vi "VHistFile - Open or Create File.vi"(6 "create if doesn't exist (F)":bool, 8 "error in":errorcluster, 9 "deny mode (2)":T1(ring)=enum."deny none", 10 "open mode (0)":T2(ring), 11 "file path":path) -> (0 "error out":errorcluster, 3 "file refnum":refnum<file>)   [LabVIEW 2021]
doc: "::: CalcExpress Toolkit :::\nCopyright (c) 2000-2026 Konstantin Shifershteyn. All rights reserved."
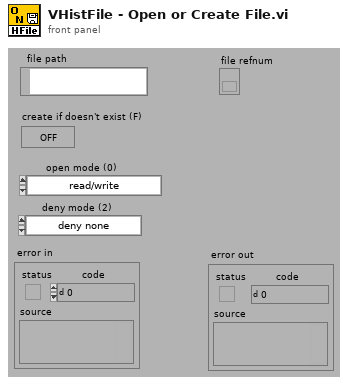
[diagram p1: front panel]
types:
  T1 = enum16{"deny read/write", "deny write-only", "deny none"}
  T2 = enum16{"read/write", "read-only", "write-only", "write-only (truncate)"}
  T3 = enum16{"open", "replace", "create", "open or create", "replace or create", "replace or create with confirmation"}
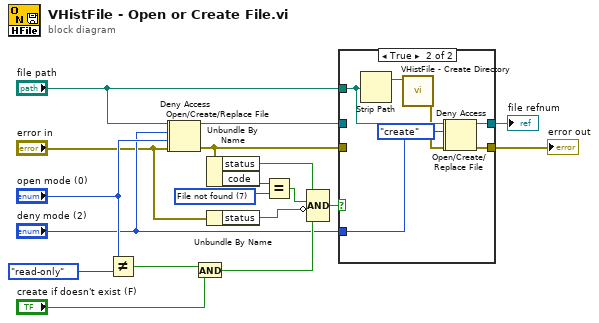
[diagram p0: block diagram]
diagram:
  w15 = u16 7 items=["No error", "Argument error", "Memory is full", "Out of zone", "End of file", "File already open", "Generic file I/O error", "File not found", "File permission error", "Disk is full", "Duplicate path", "Too many files open", "System feature not enabled", "Resource file not found", "Cannot add resource", "Resource not found", "Image not found", "Image memory error", "Pen does not exist", "Config type invalid", "Config token not found", "Config parse error", "Config memory error", "Bad external code format", "Bad external code offset", "External code not present", "Null window", "Destroy window error", "Null menu", "Print aborted", "Bad print record", "Print driver error", "Windows error during printing", "Memory error during printing", "Print dialog error", "Generic print error", "Invalid device refnum", "Device not found", "Device parameter error", "Device unit error", "Cannot open device", "Device call aborted", "Generic error", "Cancelled by user", "Object ID too low", "Object ID too high", "Object not in heap", "Unknown heap", "Unknown object (invalid DefProc)", "Unknown object (DefProc not in table)", "Message out of range", "Invalid (null) method", "Unknown message", "Manager call not supported", "Bad address", "Network operation in progress", "Network operation timed out", "Connection is busy", "Network attribute not supported", "Network error", "Address in use", "System out of memory", "Connection aborted", "Connection refused", "Not connected", "Already connected", "Connection closed", "Initialization error (interapplication manager)", "Bad occurrence", "Wait on unbound occurrence handler", "Occurrence queue overflow", "Datalog type conflict", "Unused", "Unrecognized type (interapplication manager)", "Memory corrupt", "Failed to make temporary DLL", "Old CIN version", "Drag socket not found", "Failed to load drop-object", "Failed to register OLE object", "Failed to release OLE object", "Format specifier type mismatch", "Unknown format specifier", "Too few format specifiers", "Too many format specifiers", "Scan failed", "Newer CIN version", "OLE Convert", "Runtime menu error", "Password tampered", "Unknown error code"]
  n1 = Not Equal?(x="open mode (0)", y=T2."read-only") -> (x != y?=w19:bool)
  n2 = Open/Create/Replace File(file path (use dialog)="file path", error in="error in", access (0:read/write)="open mode (0)") -> (refnum out=w1:refnum<file>, error out=w2:errorcluster)  [unwired: 3 in, 1 out]
  n3 = Deny Access(4:w2, 6:"deny mode (2)", 7:w1) -> (0:w11:errorcluster, 3:w10:refnum<file>)
  n4 = And(x=w19, y="create if doesn't exist (F)") -> (x .and. y?=w20:bool)
  n5 = Unbundle By Name(w11) -> ("status"=w12:bool, "code"=w16:i32)
  n6 = Unbundle By Name("error in") -> ("status"=w4:bool)
  n7 = Equal?(x=w16, y=w15) -> (x = y?=w17:bool)
  n8 = Compound Arithmetic op=AND(w12, w17, invert w4, w20) -> (w8:bool)
  n9 = case shown="True" w8 {
    tunnel: w10 -> [w22 _]
    tunnel: w11 -> [w21 _]
    tunnel: "deny mode (2)" -> [_ w26]
    tunnel: [w22 w30] -> w7
    tunnel: [w21 w29] -> w6
    tunnel: "file path" -> [_ w28]
    frame False {
    }
    frame True {
      n10 = Strip Path(path=w28) -> (stripped path=w31:path)  [unwired: 1 out]
      n11 = call "VHistFile - Create Directory.vi"("directory path"=w31) -> ("error out"=w27:errorcluster)  [unwired: 6 in, 2 out]
      n12 = Open/Create/Replace File(file path (use dialog)=w28, error in=w27, operation (0:open)=T3."create") -> (refnum out=w24:refnum<file>, error out=w25:errorcluster)  [unwired: 3 in, 1 out]
      n13 = Deny Access(4:w25, 6:w26, 7:w24) -> (0:w29:errorcluster, 3:w30:refnum<file>)
    }
  }
  "error out" <- w6
  "file refnum" <- w7
